vi "DAC Init Results.vi"(8 "error in":errorcluster, 9 "Log Details?":bool, 10 "tdms file":refnum<k34>, 11 "DAC CS Humid in":refnum<class "DAC CS Humid.lvclass">) -> (0 "error out":errorcluster, 2 "tdms file out":refnum<k34>)   [LabVIEW 2019, in "DAC.lvlib" / "DAC CS Humid.lvclass"]
uses:
  DAC CS Humid.lvclass
  C:/Users/krio/Documents/LV_Projects/test-stand/App/DAC/DAC.lvclass
  DAC.lvclass/DAC.ctl
  DAC CS Humid.lvclass/DAC CS Humid.ctl
  DAC.lvclass
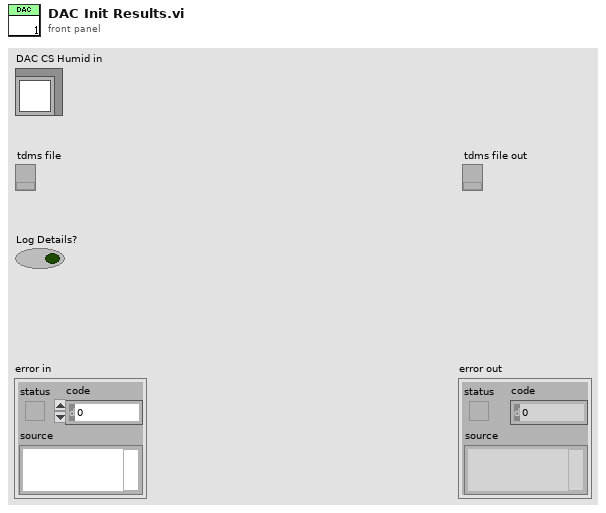
[diagram p1: front panel]
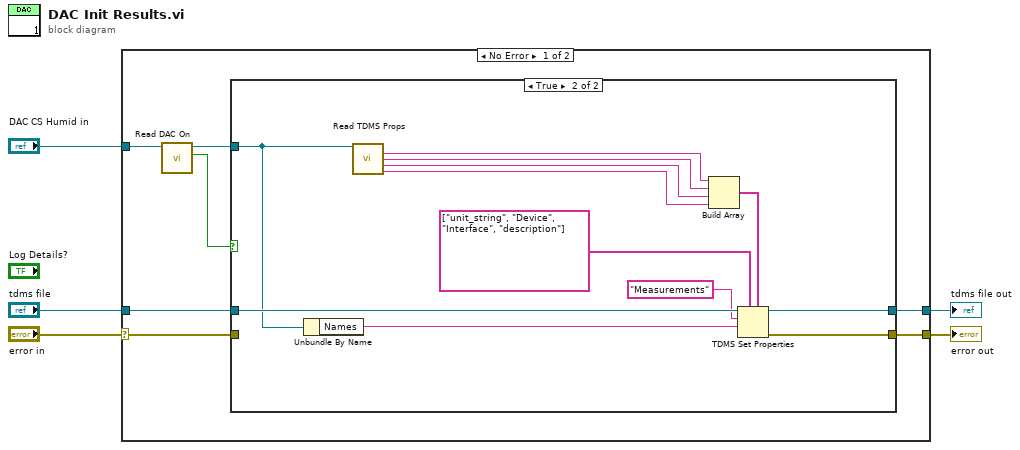
[diagram p0: block diagram]
diagram:
  n1 = case shown="No Error" "error in" {
    selector: "error in" -> [w7 w28]
    tunnel: [w10 w28] -> w2
    tunnel: "DAC CS Humid in" -> [w9 _]
    tunnel: "tdms file" -> [w12 w27]
    tunnel: [w11 w27] -> w1
    frame No Error {
      n2 = call "Read DAC On.vi"("DAC in"=w9) -> ("DAC On"=w6:bool, "DAC out"=w8:refnum<class "DAC CS Humid.lvclass">)  [unwired: 8 in, 1 out]
      n3 = case shown="True" w6 {
        tunnel: w12 -> [w14 w26]
        tunnel: [w14 w25] -> w11
        tunnel: [w13 w24] -> w10
        tunnel: w8 -> [_ w21]
        tunnel: w7 -> [w13 _]
        frame False {
        }
        frame True {
          n4 = Unbundle By Name(w21) -> ("Names"=w15:string)
          n5 = call "Read TDMS Props.vi"("DAC in"=w21) -> ("Result Unit"=w20:string, "DAC Device"=w19:string, "DAC IO"=w18:string, "DAC Description"=w17:string)  [unwired: 10 in, 1 out]
          n6 = Build Array(w20, w19, w18, w17) -> (w23:string[])
          n7 = TDMS Set Properties(5:w23, 7:string[] ["unit_string", "Device", "Interface", "description"] ("property names"), 9:w15, 10:"Measurements" ("group name in (Untitled)"), 11:w26) -> (0:w24:errorcluster, 3:w25:refnum<k34>)  [unwired: 1 in, 2 out]
        }
      }
    }
    frame Error {
    }
  }
  "error out" <- w2
  "tdms file out" <- w1
